vi "Write.vi"(8 "error in (no error)":errorcluster, 10 "data":string, 11 "pipe writer in":refnum<data-value>) -> (0 "error out":errorcluster, 1 "bytes written":i32, 2 "data out":string, 3 "pipe writer out":refnum<data-value>)   [LabVIEW 2016, in "Linux RT IPC.Pipes.lvlib" / "Unix Pipe Writer.lvclass"]
doc: "This VI writes a certain number of bytes to the provided pipe endpoint."
uses:
  Unix Pipe Writer.lvclass
  C:/Git/SourceTree/LinuxRT-IPC/Source/Pipes/Classes/Unix Pipe/Unix Pipe.lvclass
  Unix Pipe/Unix Pipe.lvclass/Unix Pipe.ctl
  C/SubVIs/error handler.vi
  <vilib>/NI/NI Linux RT Errno/VIs/Public/Get Errno Value for Calling Thread.vi
  Unix Pipe/Unix Pipe.lvclass
  C/Linux RT IPC.C.lvlib
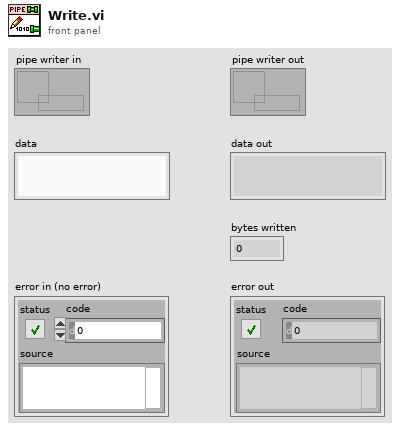
[diagram p1: front panel]
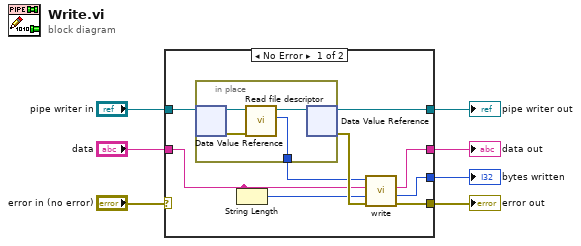
[diagram p0: block diagram]
diagram:
  n1 = case shown="No Error" "error in (no error)" {
    selector: "error in (no error)" -> [_ w22]
    tunnel: "pipe writer in" -> [w16 w23]
    tunnel: [w15 w23] -> w5
    tunnel: [w13 w22] -> w4
    tunnel: [w11 _] -> w3
    tunnel: "data" -> [w10 w21]
    tunnel: [w8 w21] -> w1
    frame No Error {
      n2 = in-place {
        in-place-border: [w18] -> w12
        n3 = in-place-dvr #1(w16) -> (w20:refnum<class "Unix Pipe Writer.lvclass">, w19:errorcluster)
        n4 = call "Read file descriptor.vi"("error in (no error)"=w19, "Unix Pipe in"=w20) -> ("file descriptor"=w18:i32, "Unix Pipe out"=w17:refnum<class "Unix Pipe Writer.lvclass">)  [unwired: 7 in, 1 out]
        n5 = in-place-dvr #1(w17) -> (w15:refnum<data-value>, w14:errorcluster)
      }
      n6 = String Length(string=w10) -> (length=w9:i32)
      n7 = call "write.vi"("error in (no error)"=w14, "bytes to write"=w9, "data"=w10, "file descriptor in"=w12) -> ("error out"=w13:errorcluster, "bytes written"=w11:i32, "data out"=w8:string)  [unwired: 4 in, 1 out]
    }
    frame Error {
    }
  }
  "error out" <- w4
  "pipe writer out" <- w5
  "bytes written" <- w3
  "data out" <- w1
